vi "Test TCPConnection Process Kill.vi"() -> ()   [LabVIEW 2013]
uses:
  <vilib>/LabVIEW Open Source Project/Connection/Connection/Connection.lvclass
panel:
  out "connected":bool
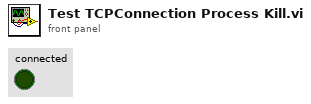
[diagram p1: front panel]
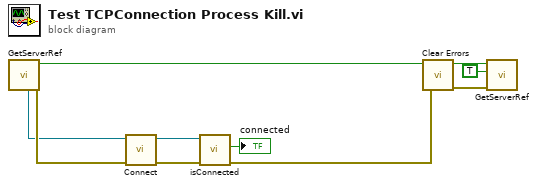
[diagram p0: block diagram]
diagram:
  n1 = call "GetServerRef.vi"() -> ("error out"=w7:errorcluster, "Created"=w9:bool, "Connection Config"=w5:refnum<class "Connection.lvclass">)  [unwired: 8 in, 1 out]
  n2 = call <vilib>:"Connect.vi"("error in (no error)"=w7, "Connection in"=w5) -> ("error out"=w3:errorcluster, "Connection out"=w4:refnum<class "Connection.lvclass">)  [unwired: 8 in]
  n3 = call <vilib>:"isConnected.vi"("error in (no error)"=w3, "Connection in"=w4) -> ("error out"=w1:errorcluster, "connected"=→"connected":bool)  [unwired: 7 in, 1 out]
  n4 = call <vilib>:"Clear Errors.vi"("error in (no error)"=w1) -> ("error out"=w6:errorcluster)  [unwired: 6 in]
  n5 = call "GetServerRef.vi"("error in"=w6, "Force Destroy (F)"=TRUE, "Destroy (F)"=w9) -> ()  [unwired: 5 in, 4 out]
